vi "Scripting_UpdateBundle.vi"(8 "error in (no error)":errorcluster, 9 "Boolean":bool, 10 "PropertyName":string, 11 "VI in":refnum<vi>) -> (0 "error out":errorcluster)   [LabVIEW 2020]
panel:
  out "Full Element Names[]":cluster{string[]}[](array[cluster])
  out "Element Names[]":string[](array[string])
  out "Available Elements[]":string[](array[string])
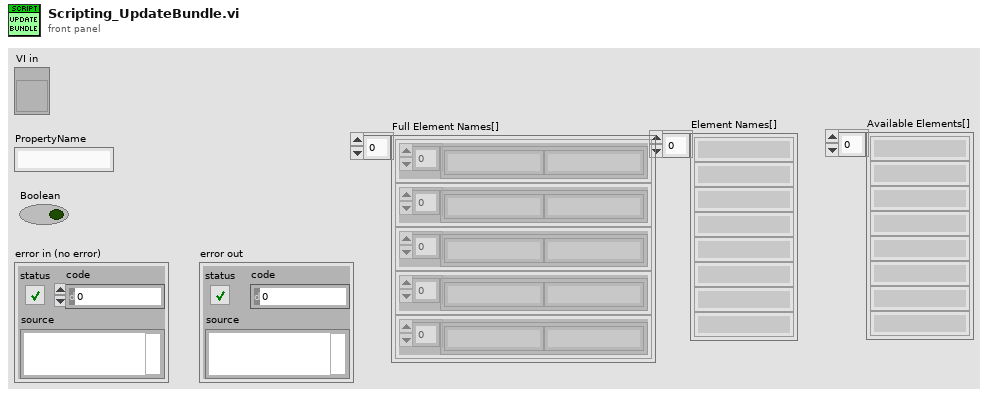
[diagram p1: front panel]
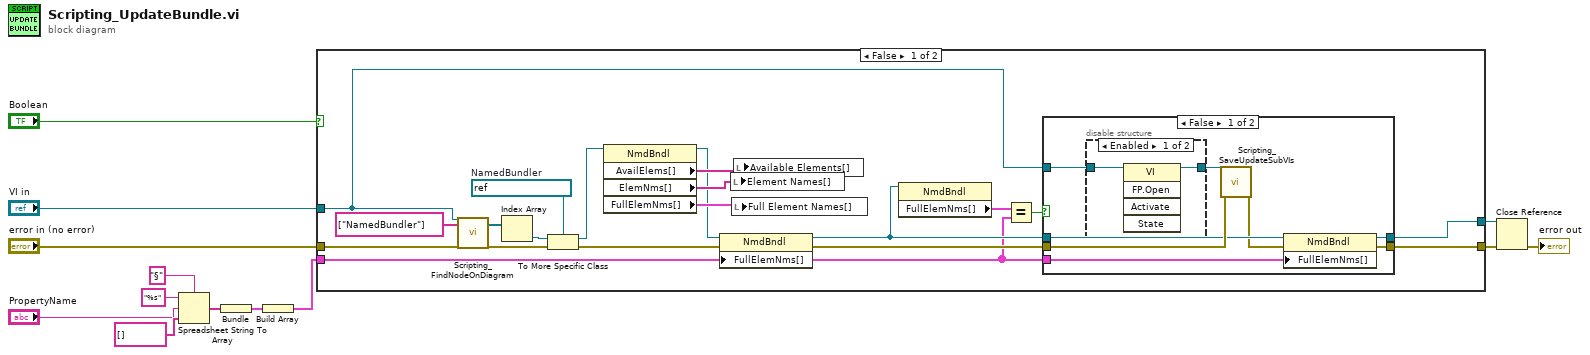
[diagram p0: block diagram]
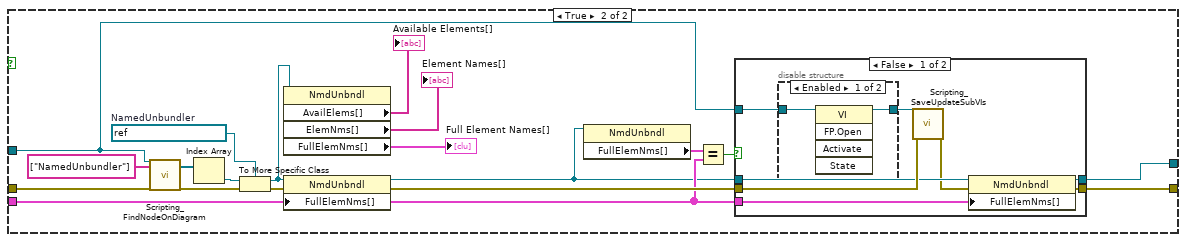
[diagram p4: hidden frame]
diagram:
  n1 = Spreadsheet String To Array(delimiter (Tab)="§" ("search string"), format string="%s", spreadsheet string="PropertyName", array type (2D Dbl)=string[] [] ("appended array")) -> (array=w10:string[])
  n2 = Bundle("appended array"=w10) -> (w6:cluster{"appended array":string[]})  [unwired: 1 in]
  n3 = Build Array(w6) -> (w7:cluster{"appended array":string[]}[])
  n4 = case shown="False" "Boolean" {
    tunnel: "error in (no error)" -> [w29 w62]
    tunnel: "VI in" -> [w20 w46]
    tunnel: w7 -> [w18 w48]
    tunnel: [w22 w49] -> w8
    tunnel: [w17 w50] -> w9
    frame False {
      w14 = refnum<vi> refnum  # NamedBundler
      n5 = call "Scripting_FindNodeOnDiagram.vi"("ViRef(Ignored If Not Wired)"=w20, "NodeTypesToSearchFor"=string[] ["NamedBundler"], "error in (no error)"=w29) -> ("Nodes"=w30:refnum<vi>[], "error out"=w33:errorcluster)  [unwired: 15 in]
      n6 = Index Array(array=w30) -> (element=w32:refnum<vi>)  [unwired: 1 in]
      n7 = To More Specific Class(target class=w14, reference=w32, error in=w33) -> (specific class reference=w15:refnum<vi>, error out=w28:errorcluster)
      n8 = property class="NmdBndl"(reference=w15) -> (reference out=w16:refnum<vi>, "AvailElems[]"=w26:string[], "ElemNms[]"=w25:string[], "FullElemNms[]"=w27:cluster{string[]}[])  [unwired: 1 in, 1 out]
      n9 = property class="NmdBndl"(reference=w16, error in=w28, "FullElemNms[]"=w18) -> (reference out=w19:refnum<vi>, error out=w23:errorcluster)
      n10 = local write "Element Names[]"(w25) -> ()
      n11 = local write "Full Element Names[]"(w27) -> ()
      n12 = local write "Available Elements[]"(w26) -> ()
      n13 = property class="NmdBndl"(reference=w19) -> ("FullElemNms[]"=w24:cluster{string[]}[])  [unwired: 1 in, 2 out]
      n14 = Equal?(x=w24, y=w18) -> (x = y?=w21:bool)
      n15 = case shown="False" w21 {
        tunnel: w23 -> [w40 w45]
        tunnel: [w36 w45] -> w22
        tunnel: w20 -> [w39 _]
        tunnel: w19 -> [w37 w44]
        tunnel: w18 -> [w35 _]
        tunnel: [w34 w44] -> w17
        frame False {
          n16 = disable-structure shown="Enabled" {
            disable-tunnel: w39 -> [w42 w43]
            disable-tunnel: [w41 w43] -> w38
            frame Enabled {
              n17 = invoke class="VI" method="FP.Open"(reference=w42) -> (reference out=w41:refnum<vi>)  [unwired: 4 in, 4 out]
            }
            frame Disabled {
            }
          }
          n18 = call "Scripting_SaveUpdateSubVIs.vi"("error in (no error)"=w40, "VI Refnum"=w38) -> ("error out"=w36:errorcluster)  [unwired: 9 in]
          n19 = property class="NmdBndl"(reference=w37, error in=w36, "FullElemNms[]"=w35) -> (reference out=w34:refnum<vi>)  [unwired: 1 out]
        }
        frame True {
        }
      }
    }
    frame True {
      w58 = refnum<vi> refnum  # NamedUnbundler
      n20 = call "Scripting_FindNodeOnDiagram.vi"("ViRef(Ignored If Not Wired)"=w46, "NodeTypesToSearchFor"=string[] ["NamedUnbundler"], "error in (no error)"=w62) -> ("Nodes"=w63:refnum<vi>[], "error out"=w61:errorcluster)  [unwired: 15 in]
      n21 = Index Array(array=w63) -> (element=w60:refnum<vi>)  [unwired: 1 in]
      n22 = To More Specific Class(target class=w58, reference=w60, error in=w61) -> (specific class reference=w57:refnum<vi>, error out=w59:errorcluster)
      n23 = property class="NmdUnbndl"(reference=w57) -> ("AvailElems[]"=→"Available Elements[]":string[], "ElemNms[]"=→"Element Names[]":string[], "FullElemNms[]"=→"Full Element Names[]":cluster{string[]}[])  [unwired: 1 in, 2 out]
      n24 = property class="NmdUnbndl"(reference=w57, error in=w59, "FullElemNms[]"=w48) -> (reference out=w47:refnum<vi>, error out=w51:errorcluster)
      n25 = property class="NmdUnbndl"(reference=w47) -> ("FullElemNms[]"=w53:cluster{string[]}[])  [unwired: 1 in, 2 out]
      n26 = Equal?(x=w53, y=w48) -> (x = y?=w52:bool)
      n27 = case shown="False" w52 {
        tunnel: w51 -> [w71 w76]
        tunnel: [w67 w76] -> w49
        tunnel: w46 -> [w70 _]
        tunnel: w47 -> [w68 w75]
        tunnel: w48 -> [w66 _]
        tunnel: [w65 w75] -> w50
        frame False {
          n28 = disable-structure shown="Enabled" {
            disable-tunnel: w70 -> [w73 w74]
            disable-tunnel: [w72 w74] -> w69
            frame Enabled {
              n29 = invoke class="VI" method="FP.Open"(reference=w73) -> (reference out=w72:refnum<vi>)  [unwired: 4 in, 4 out]
            }
            frame Disabled {
            }
          }
          n30 = call "Scripting_SaveUpdateSubVIs.vi"("error in (no error)"=w71, "VI Refnum"=w69) -> ("error out"=w67:errorcluster)  [unwired: 9 in]
          n31 = property class="NmdUnbndl"(reference=w68, error in=w67, "FullElemNms[]"=w66) -> (reference out=w65:refnum<vi>)  [unwired: 1 out]
        }
        frame True {
        }
      }
    }
  }
  n32 = Close Reference(reference=w9, error in (no error)=w8) -> (error out=→"error out":errorcluster)
